vi "Test Confluence VIDoc.vi"() -> ()   [LabVIEW 2023]
uses:
  <userlib>/_PetranWay/LabVIEW Confluence API/Source/Confluence/Confluence Connection/Confluence.lvclass
  <userlib>/_PetranWay/LabVIEW Confluence API/Source/Cloud/Confluence Cloud/Confluence Cloud.lvclass
  C:/Program Files/National Instruments/LabVIEW 2023/user.lib/_PetranWay/LabVIEW Confluence API/Source/Confluence/Confluence Connection/Confluence.lvclass
  <vilib>/DMC/VIDoc/Framework/UI Interaction/Progress Bar UI/Progress Bar UI.lvclass
  C:/Program Files/National Instruments/LabVIEW 2023/vi.lib/DMC/VIDoc/Framework/UI Interaction/Interface/UI Interaction.lvclass
  <userlib>/_PetranWay/LabVIEW Confluence API/Source/Cloud/Confluence Cloud/API/Construct Confluence Cloud From Cache.vi
  Source/Confluence Printer/VIDoc Printer - Confluence.lvclass
  <vilib>/DMC/VIDoc/Framework/Parsing/Documentation Parser/VIDoc Parser.lvclass
panel:
  in  "Tab Control":enum32{"Use Settings File", "Cloud Connection"}(tab)
  in  "Organization Name":string caption="Organization Name (https://[Organization Name].atlassian.net]"
  in  "Email Address":string
  in  "Top Page ID":string
  in  "Source Root":path
  in  "VIDoc json Settings Path":path
  out "Group":string
  out "Section":string
  out "error out":errorcluster {"code" format="Error %.0f"}
  out "Message":string
  out "Progress Bar":i32(slide) max=28 scale=0.0..7.0
  in  "Abort":bool
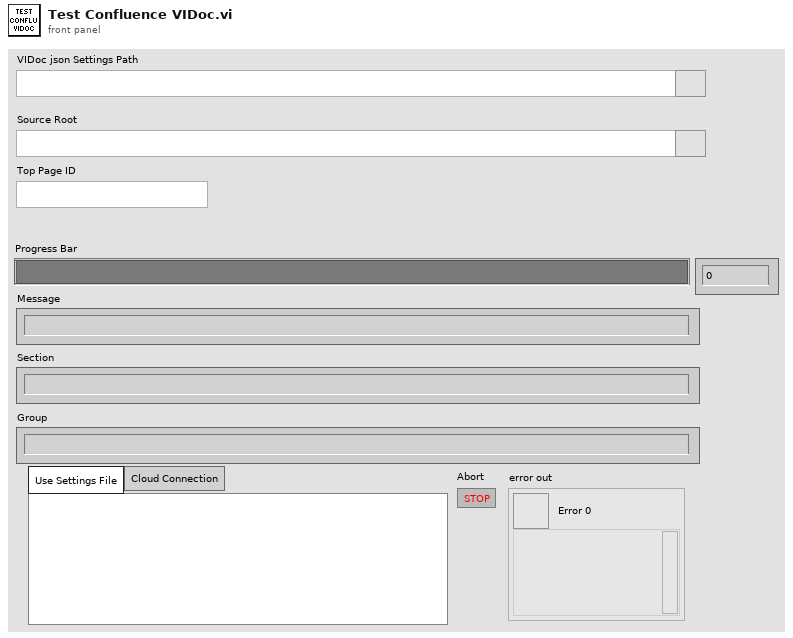
[diagram p1: front panel]
types:
  T1 = cluster{"Progress Max":refnum<user-event>, "Progress Value":refnum<user-event>, "Message":refnum<user-event>, "Stopped":refnum<user-event>, "Section":refnum<user-event>, "Group":refnum<user-event>}
  T2 = typedef "VIDoc Parsing.lvlib/Full Documentation Info.ctl" = cluster{"Projects":refnum<class "Project Documentation.lvclass">[], "Interfaces":refnum<class "Interface Documenation.lvclass">[], "Classes":refnum<class "Class Documentation.lvclass">[], "Libraries":refnum<class "Library Documentation.lvclass">[], "VI Members":refnum<class "GUI Documentation.lvclass">[], "Controls":refnum<class "GUI Documentation.lvclass">[], "LLBs":refnum<class "LLB Documentation.lvclass">[], "Bookmarked Map":map{string, refnum<class "GUI Documentation.lvclass">[]}}
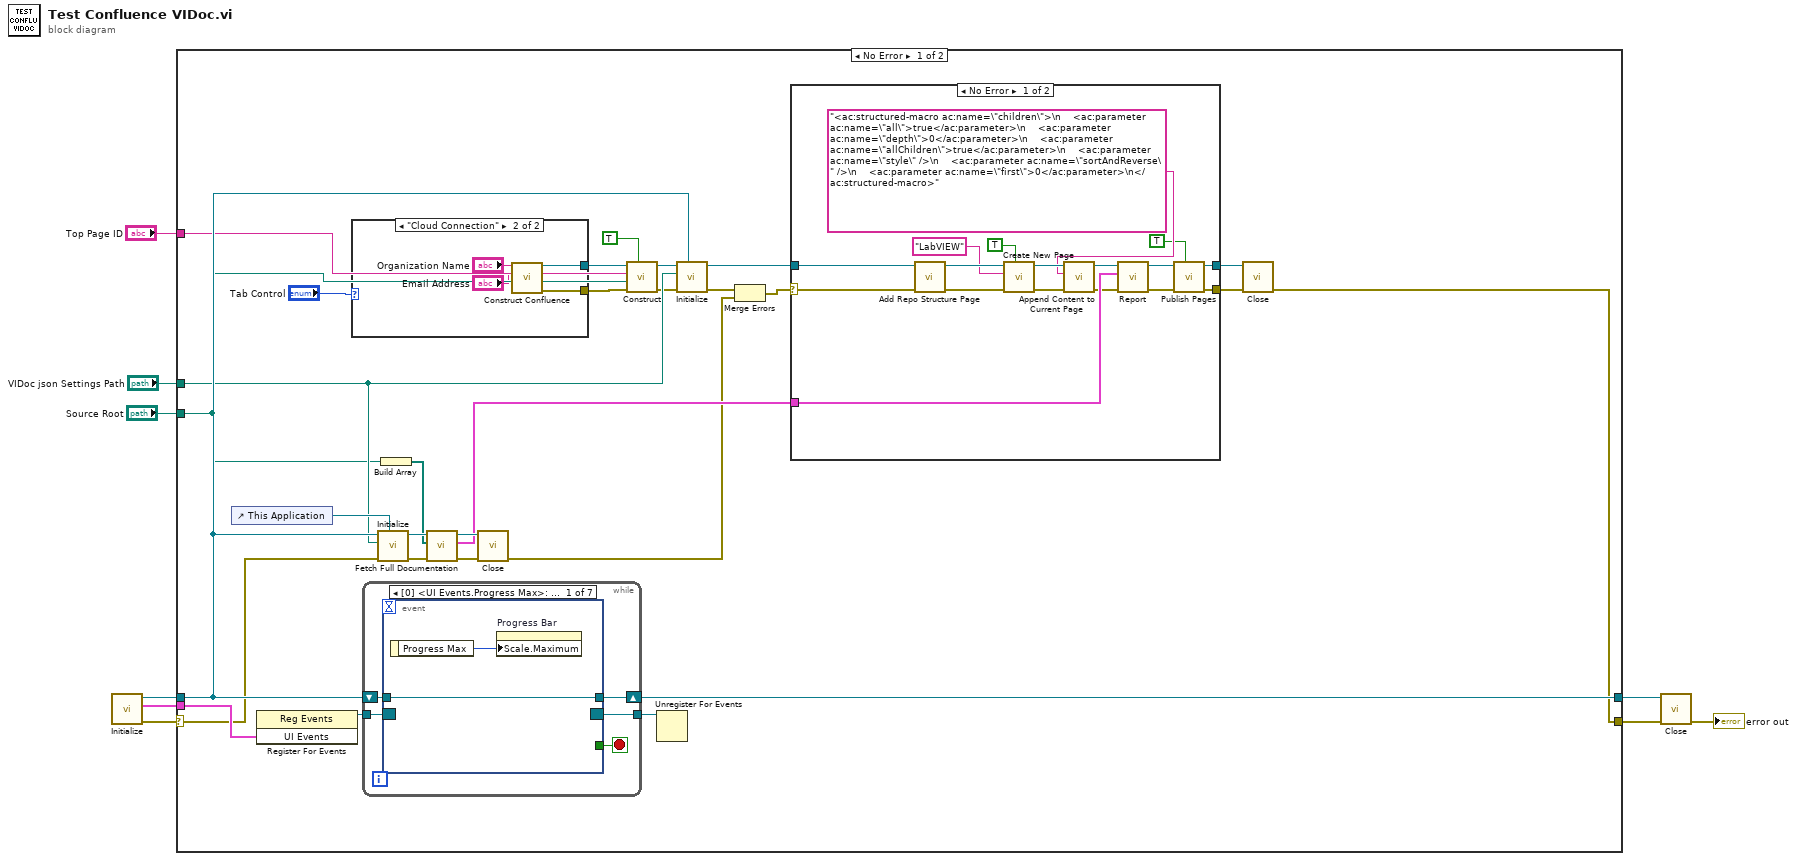
[diagram p0: block diagram]
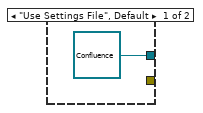
[diagram p2: hidden frame]
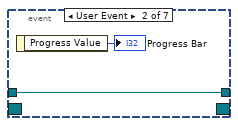
[diagram p4: hidden frame]
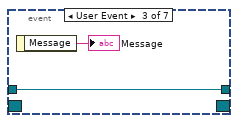
[diagram p5: hidden frame]
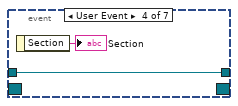
[diagram p6: hidden frame]
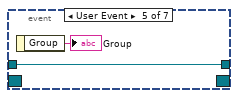
[diagram p7: hidden frame]
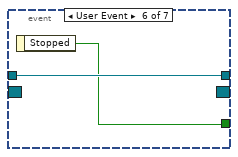
[diagram p8: hidden frame]
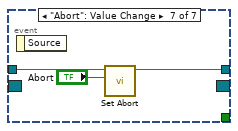
[diagram p9: hidden frame]
diagram:
  n1 = call <vilib>:"Initialize.vi"() -> ("error out"=w6:errorcluster, "UI Events"=w9:T1, "Progress Bar UI Out"=w7:refnum<class "Progress Bar UI.lvclass">)  [unwired: 9 in]
  n2 = case shown="No Error" w6 {
    selector: w6 -> [w26 w84]
    tunnel: w9 -> [w38 _]
    tunnel: [w36 w83] -> w8
    tunnel: w7 -> [w35 w83]
    tunnel: [w30 w84] -> w5
    tunnel: "VIDoc json Settings Path" -> [w25 _]
    tunnel: "Source Root" -> [w24 _]
    tunnel: "Top Page ID" -> [w23 _]
    frame No Error {
      n3 = control-ref of="This Application"() -> (w27:refnum<vi>)
      n4 = register-events(w38) -> (reference out=w37:refnum<event-registration>)  [unwired: 2 in, 1 out]
      n5 = case shown="\"Cloud Connection\"" "Tab Control" {
        tunnel: [refnum<class "Confluence.lvclass"> refnum ("Confluence") w41] -> w12
        tunnel: [_ w40] -> w11
        frame "Use Settings File", Default {
        }
        frame "Cloud Connection" {
          n6 = call-poly <userlib>:"Construct Confluence.vi"("Organization Name (https://[Organization Name].atlassian.net]"="Organization Name", "Email Address"="Email Address") -> ("Confluence Cloud out"=w41:refnum<class "Confluence Cloud.lvclass">, "error out"=w40:errorcluster)  [unwired: 10 in, 2 out]
        }
      }
      n7 = while {
        tunnel: w37 -> [w67]
        shift-right: [w65] -> w36
        shift-left: w35 -> [w66]
        tunnel: [w63] -> w22
        stop <- w64 stop-if-true
        n8 = event shown="[0] <UI Events.Progress Max>: User Event" {
          selector: w67 -> [_ _ _ _ _ _ _]
          dyn-events: [_ _ _ _ _ _ _] -> w63
          timeout: _ -> [_ _ _ _ _ _ _]
          tunnel: w66 -> [w69 w71 w73 w75 w77 w79 w81]
          tunnel: [w69 w71 w73 w75 w77 w79 w82] -> w65
          tunnel: [_ _ _ _ _ w78 _] -> w64
          event User Event {
            n9 = event-data() -> ("Progress Max"=w68:i32)  [unwired: 1 in]
            n10 = property on="Progress Bar" class="Slide (strict)"("Scale.Maximum"=w68) -> ()  [unwired: 2 in, 2 out]
          }
          event User Event {
            n11 = event-data() -> ("Progress Value"=→"Progress Bar":i32)  [unwired: 1 in]
          }
          event User Event {
            n12 = event-data() -> ("Message"=→"Message":string)  [unwired: 1 in]
          }
          event User Event {
            n13 = event-data() -> ("Section"=→"Section":string)  [unwired: 1 in]
          }
          event User Event {
            n14 = event-data() -> ("Group"=→"Group":string)  [unwired: 1 in]
          }
          event User Event {
            n15 = event-data() -> ("Stopped"=w78:bool)  [unwired: 1 in]
          }
          event "Abort": Value Change {
            n16 = event-data() -> ()  [unwired: 1 in, 1 out]
            n17 = call <vilib>:"Set Abort.vi"("Abort?"="Abort", "Progress Bar UI In"=w81) -> ("Progress Bar UI Out"=w82:refnum<class "Progress Bar UI.lvclass">)  [unwired: 8 in, 1 out]
          }
        }
      }
      n18 = call <vilib>:"Initialize.vi"("App Reference (This Application)"=w27, "error in (no error)"=w26, "Settings Path"=w25, "UI Interaction"=w35) -> ("error out"=w34:errorcluster, "VIDoc Parser Out"=w33:refnum<class "VIDoc Parser.lvclass">)  [unwired: 6 in]
      n19 = Build Array(w24) -> (w28:path[])
      n20 = call <vilib>:"Fetch Full Documentation.vi"("error in (no error)"=w34, "File Paths"=w28, "VIDoc Parser In"=w33) -> ("error out"=w31:errorcluster, "Full Documentation"=w29:T2, "VIDoc Parser Out"=w32:refnum<class "VIDoc Parser.lvclass">)  [unwired: 6 in]
      n21 = call <vilib>:"Close.vi"("error in (no error)"=w31, "VIDoc Parser In"=w32) -> ("error out"=w13:errorcluster)  [unwired: 9 in]
      n22 = call "Construct.vi"("Bulk Attachments? (T)"=TRUE, "error in (no error)"=w11, "Working Directory"=w24, "Top Page ID"=w23, "Confluence"=w12) -> ("error out"=w21:errorcluster, "VIDoc Printer - Confluence Out"=w20:refnum<class "VIDoc Printer - Confluence.lvclass">)  [unwired: 5 in]
      n23 = Unregister For Events(event registration refnum=w22) -> ()  [unwired: 1 in, 1 out]
      n24 = call-dynamic <vilib>:"Initialize.vi"("UI Interaction"=w35, "error in (no error)"=w21, "Settings Path"=w25, "VIDoc Printer - Confluence In"=w20) -> ("error out"=w19:errorcluster, "VIDoc Printer - Confluence Out"=w18:refnum<class "VIDoc Printer - Confluence.lvclass">)  [unwired: 6 in]
      n25 = Merge Errors(w19, w13) -> (w14:errorcluster)
      n26 = case shown="No Error" w14 {
        selector: w14 -> [w59 w61]
        tunnel: w29 -> [w60 _]
        tunnel: w18 -> [w58 w62]
        tunnel: [w57 w61] -> w16
        tunnel: [w56 w62] -> w15
        frame No Error {
          n27 = call "Add Repo Structure Page.vi"("error in (no error)"=w59, "VIDoc Printer - Confluence In"=w58) -> ("error out"=w53:errorcluster, "VIDoc Printer - Confluence Out"=w52:refnum<class "VIDoc Printer - Confluence.lvclass">)  [unwired: 8 in]
          n28 = call "Create New Page.vi"("Update Current Page (F)"=TRUE, "error in (no error)"=w53, "Name"="LabVIEW", "VIDoc Printer - Confluence In"=w52) -> ("error out"=w47:errorcluster, "VIDoc Printer - Confluence Out"=w49:refnum<class "VIDoc Printer - Confluence.lvclass">)  [unwired: 4 in, 2 out]
          n29 = call "Append Content to Current Page.vi"("error in (no error)"=w47, "Content"="<ac:structured-macro ac:name=\"children\">\n    <ac:parameter ac:name=\"all\">true</ac:parameter>\n    <ac:parameter ac:name=\"depth\">0</ac:parameter>\n    <ac:parameter ac:name=\"allChildren\">true</ac:parameter>\n    <ac:parameter ac:name=\"style\" />\n    <ac:parameter ac:name=\"sortAndReverse\" />\n    <ac:parameter ac:name=\"first\">0</ac:parameter>\n</ac:structured-macro>", "VIDoc Printer - Confluence In"=w49) -> ("error out"=w46:errorcluster, "VIDoc Printer - Confluence Out"=w48:refnum<class "VIDoc Printer - Confluence.lvclass">)  [unwired: 7 in]
          n30 = call-dynamic "Report.vi"("error in (no error)"=w46, "Full Documentation"=w60, "VIDoc Printer In"=w48) -> ("error out"=w55:errorcluster, "VIDoc Printer Out"=w54:refnum<class "VIDoc Printer - Confluence.lvclass">)  [unwired: 7 in]
          n31 = call "Publish Pages.vi"("Parallel?"=TRUE, "error in (no error)"=w55, "VIDoc Printer - Confluence In"=w54) -> ("error out"=w57:errorcluster, "VIDoc Printer - Confluence Out"=w56:refnum<class "VIDoc Printer - Confluence.lvclass">)  [unwired: 7 in]
        }
        frame Error {
        }
      }
      n32 = call-dynamic <vilib>:"Close.vi"("error in (no error)"=w16, "VIDoc Printer - Confluence In"=w15) -> ("error out"=w30:errorcluster)  [unwired: 9 in]
    }
    frame Error {
    }
  }
  n33 = call <vilib>:"Close.vi"("error in (no error)"=w5, "Progress Bar UI In"=w8) -> ("error out"=→"error out":errorcluster)  [unwired: 9 in]
